vi "Create Engine Folder and Copy RT Template.vi"(8 "error in":errorcluster, 9 "Project Root":path, 10 "Project Name":string, 11 "CD Template":refnum<class "NIVS_CD Template.lvclass">) -> (0 "error out":errorcluster)   [LabVIEW 2020, in "NIVS_CD Template.lvclass"]
uses:
  NIVS_CD Template.lvclass
  NIVS_Consolidated_CDW_MetaDataObj/CD Engine lvlib.ctl
  NIVS_CD Template.lvclass/NIVS_CD Template.ctl
  NIVS_Consolidated_CDW_MetaDataObj/Common.ctl
  NIVS_Consolidated_CDW_MetaDataObj/Common.vi
  NIVS_Consolidated_CDW_MetaDataObj/NIVS_Consolidated_CDW_MetaDataObj.lvclass
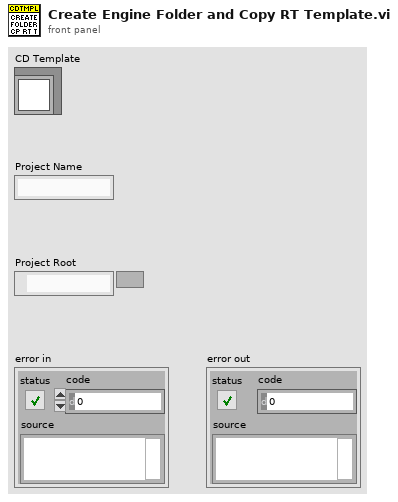
[diagram p1: front panel]
types:
  T1 = typedef "NIVS_Consolidated_CDW_MetaDataObj.lvclass/CD Engine lvlib.ctl" = enum16{"LibraryFileName", "LibraryFolderName", "Engine.FolderName", "Engine.Init.FolderName", "Engine.Run.FolderName", "Engine.Shutdown.FolderName", "Types.FolderName", "Engine.RT Driver VI.TemplatePath", "Engine.RT Driver VI.FileName", "Engine.PPL.RT Driver VI_InlineAsync.FileName", "Engine.RTStateVariables.Name", "Engine.PPL.RTStateVariables.Name", "Engine.RTStateVariables.Name.NoExtension", "Engine.Async.NameExtension", "Engine.Async.TemplateName", "Engine.PPL.Async.TemplateName", "Engine.PPL.Async.InitVSGlobals.Name", "Engine.PPL.RT Driver VI_Inline.FileName", "Engine.LaunchCommandLoop.Name", "Engine.CommandLoop.Name"}
  T2 = typedef "NIVS_Consolidated_CDW_MetaDataObj.lvclass/Common.ctl" = enum16{"ProjectName", "TemplatesFolderName", "PPLTemplatesFolderName", "ProjectTemplatePathAndName", "ProjectPPLTemplatePathAndName", "TimingAndSyncFolderName", "CustomDeviceFolderName", "PathToTemplates", "PathToPPLTemplates", "PathToExplorerPPLTemplates", "PathToEnginePPLTemplates", "PathToConfigurationFile", "ProjectConfigurationName"}
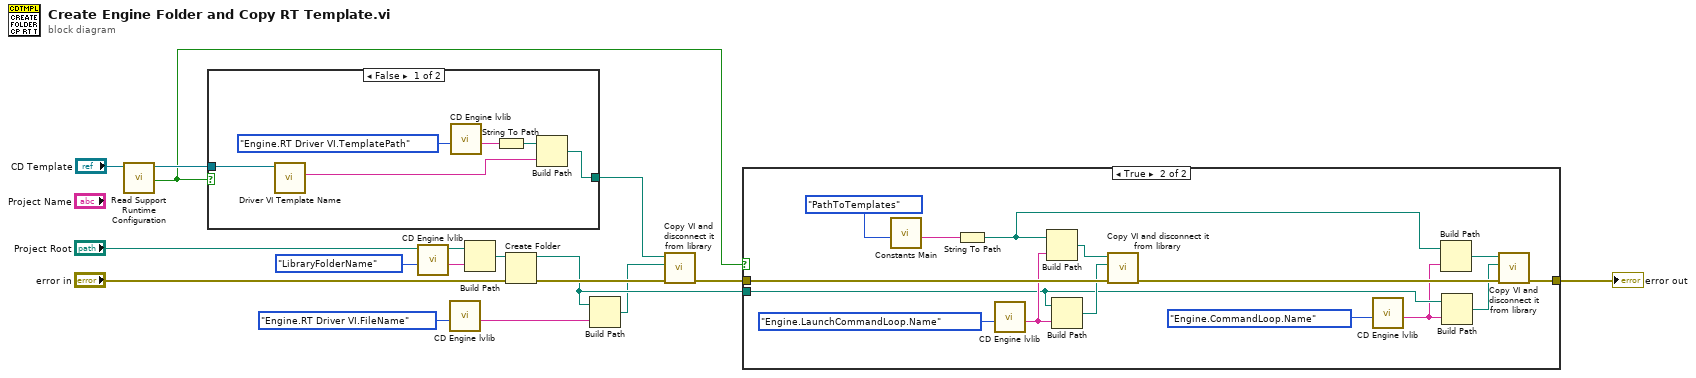
[diagram p0: block diagram]
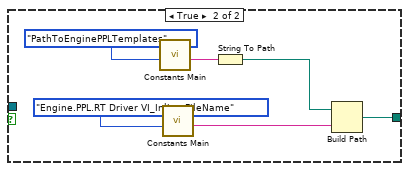
[diagram p2: hidden frame]
diagram:
  n1 = call "Read Support Runtime Configuration.vi"("NIVS_CD Template in"="CD Template") -> ("Support Runtime Configuration"=w2:bool)  [unwired: 8 in, 2 out]
  n2 = case shown="False" w2 {
    tunnel: "CD Template" -> [w21 _]
    tunnel: [w16 w22] -> w1
    frame False {
      n3 = call-dynamic "Driver VI Template Name.vi"("CD Template"=w21) -> ("Driver VI Template Name"=w18:string)  [unwired: 10 in]
      n4 = call "CD Engine lvlib.vi"("Action"=CD_Engine_lvlib."Engine.RT Driver VI.TemplatePath") -> ("Output"=w20:string)  [unwired: 10 in]
      n5 = String To Path(string=w20) -> (path=w19:path)
      n6 = Build Path(base path=w19, name or relative path=w18) -> (appended path=w16:path)
    }
    frame True {
      n7 = call-poly "Constants Main.vi"("Action"=Common."PathToEnginePPLTemplates") -> ("Output"=w26:string)  [unwired: 10 in]
      n8 = call-poly "Constants Main.vi"("Action"=CD_Engine_lvlib."Engine.PPL.RT Driver VI_Inline.FileName") -> ("Output"=w24:string)  [unwired: 10 in]
      n9 = String To Path(string=w26) -> (path=w25:path)
      n10 = Build Path(base path=w25, name or relative path=w24) -> (appended path=w22:path)
    }
  }
  n11 = call "CD Engine lvlib.vi"("Action"=CD_Engine_lvlib."LibraryFolderName") -> ("Output"=w7:string)  [unwired: 10 in]
  n12 = call "CD Engine lvlib.vi"("Action"=CD_Engine_lvlib."Engine.RT Driver VI.FileName") -> ("Output"=w8:string)  [unwired: 10 in]
  n13 = Build Path(base path="Project Root", name or relative path=w7) -> (appended path=w6:path)
  n14 = Create Folder(path (use dialog)=w6, error in="error in") -> (created path=w5:path, error out=w15:errorcluster)  [unwired: 1 in, 1 out]
  n15 = Build Path(base path=w5, name or relative path=w8) -> (appended path=w4:path)
  n16 = call "Copy VI and disconnect it from library.vi"("error in (no error)"=w15, "VI Target Path"=w4, "VI Source Path"=w1) -> ("error out"=w13:errorcluster)  [unwired: 8 in]
  n17 = case shown="True" w2 {
    tunnel: w13 -> [w28 w43]
    tunnel: [w28 w41] -> w12
    tunnel: w5 -> [_ w33]
    frame False {
    }
    frame True {
      n18 = call-poly "Constants Main.vi"("Action"=Common."PathToTemplates") -> ("Output"=w36:string)  [unwired: 10 in]
      n19 = String To Path(string=w36) -> (path=w30:path)
      n20 = call "CD Engine lvlib.vi"("Action"=CD_Engine_lvlib."Engine.LaunchCommandLoop.Name") -> ("Output"=w35:string)  [unwired: 10 in]
      n21 = Build Path(base path=w30, name or relative path=w35) -> (appended path=w37:path)
      n22 = Build Path(base path=w33, name or relative path=w35) -> (appended path=w39:path)
      n23 = call "Copy VI and disconnect it from library.vi"("error in (no error)"=w43, "VI Target Path"=w39, "VI Source Path"=w37) -> ("error out"=w42:errorcluster)  [unwired: 8 in]
      n24 = call "CD Engine lvlib.vi"("Action"=CD_Engine_lvlib."Engine.CommandLoop.Name") -> ("Output"=w29:string)  [unwired: 10 in]
      n25 = Build Path(base path=w30, name or relative path=w29) -> (appended path=w31:path)
      n26 = Build Path(base path=w33, name or relative path=w29) -> (appended path=w32:path)
      n27 = call "Copy VI and disconnect it from library.vi"("error in (no error)"=w42, "VI Target Path"=w32, "VI Source Path"=w31) -> ("error out"=w41:errorcluster)  [unwired: 8 in]
    }
  }
  "error out" <- w12
